vi "Node HTTP Post.vi"(6 "Timeout ms (10000)":i32=10000, 7 "Node Name":string, 8 "error in (no error)":errorcluster, 9 "Payload":string, 10 "Path":string, 11 "VolatusAPI in":refnum<class "VolatusAPI.lvclass">) -> (0 "error out":errorcluster, 1 "Headers":string, 2 "Response":string, 3 "VolatusAPI out":refnum<class "VolatusAPI.lvclass">, 4 "Status Code":u32)   [LabVIEW 2020, in "Volatus.lvlib" / "VolatusAPI.lvclass"]
uses:
  VolatusAPI.lvclass
  VolatusAPI.lvclass/VolatusAPI.ctl
  <vilib>/httpClient/LabVIEWHTTPClient.lvlib
  <vilib>/httpClient/MultipartData.ctl
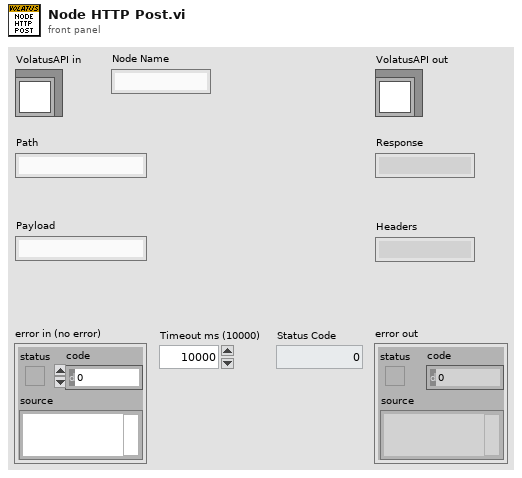
[diagram p1: front panel]
types:
  T1 = typedef "LabVIEWHTTPClient.lvlib/MultipartData.ctl" = cluster{"Name":string, "Value":string, "File":path, "Filename":string, "MIME type":string}
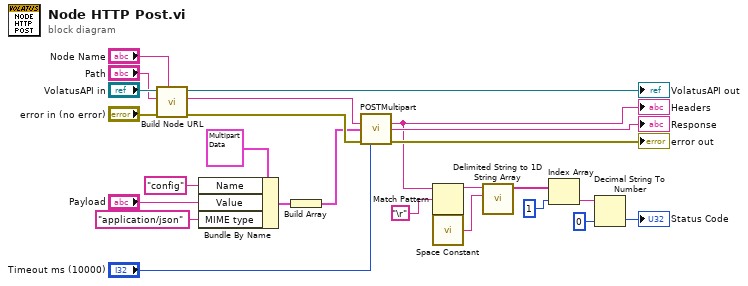
[diagram p0: block diagram]
diagram:
  n1 = call "Build Node URL.vi"("Node Name"="Node Name", "error in (no error)"="error in (no error)", "Path"="Path", "VolatusAPI in"="VolatusAPI in") -> ("error out"=w18:errorcluster, "Request URL"=w19:string, "VolatusAPI out"=→"VolatusAPI out":refnum<class "VolatusAPI.lvclass">)  [unwired: 5 in]
  n2 = Bundle By Name(cluster=T1 {"Name"="", "Value"="", "File"=path "", "Filename"="", "MIME type"="application/octet-stream"} ("Element"), "Name"="config" ("name"), "Value"="Payload", "MIME type"="application/json") -> (w12:T1)
  n3 = Build Array(w12) -> (w10:T1[])
  n4 = call <vilib>:"POSTMultipart.vi"("url"=w19, "data"=w10, "error in (no error)"=w18, "timeout (10000)"="Timeout ms (10000)") -> ("headers"=w2:string, "body"=→"Response":string, "error out"=→"error out":errorcluster)  [unwired: 8 in, 1 out]
  "Headers" <- w2
  n5 = Match Pattern(string=w2, regular expression="\r") -> (before substring=w8:string)  [unwired: 1 in, 3 out]
  n6 = call <vilib>:"Space Constant.vi"() -> ("String"=w7:string)
  n7 = call <vilib>:"Delimited String to 1D String Array.vi"("delimiter"=w7, "delimited string"=w8) -> ("string array"=w6:string[])  [unwired: 9 in]
  n8 = Index Array(array=w6, index=1) -> (element=w4:string)
  n9 = Decimal String To Number(string=w4, default (0L)=u32 0 ("default (0 I32)")) -> (number=→"Status Code":u32)  [unwired: 1 in, 1 out]
